vi "test_Set and Get 9227.vi"(8 "error in (no error)":errorcluster, 11 "TestCase in":refnum<class "Scan Engine Scripting API Custom Device Unit Tests.lvclass">) -> (0 "error out":errorcluster, 3 "TestCase out":refnum<class "Scan Engine Scripting API Custom Device Unit Tests.lvclass">)   [LabVIEW 2027, in "Scan Engine Scripting API Custom Device Unit Tests.lvclass"]
uses:
  Scan Engine Scripting API Custom Device Unit Tests.lvclass
  Scan Engine Scripting API Custom Device Unit Tests.lvclass/Scan Engine Scripting API Custom Device Unit Tests.ctl
  Scripting/Modules/NI 9227/NI 9227.lvclass
  C:/NetCore/niveristand-scan-engine-ethercat-custom-device/Custom Device Source/Scripting/Modules/Module/Module.lvclass
  C:/NetCore/niveristand-scan-engine-ethercat-custom-device/Custom Device Source/Scripting/Modules/NI 9227/NI 9227.lvclass
  C:/Program Files/National Instruments/LabVIEW 2027/vi.lib/addons/_JKI Toolkits/VI Tester/TestCase.llb/TestCase.lvclass
  C:/NetCore/niveristand-scan-engine-ethercat-custom-device/Custom Device Source/Tests/Unit Tests/Scripting API/Custom Device/Scan Engine Scripting API Custom Device Unit Tests.lvclass
  <vilib>/addons/_JKI Toolkits/VI Tester/TestCase.llb/TestCase.lvclass
  Scripting/Scan Engine Scripting.lvlib
  b7875b56-ce47-4e38-ae1e-efee4344b8b5.vi
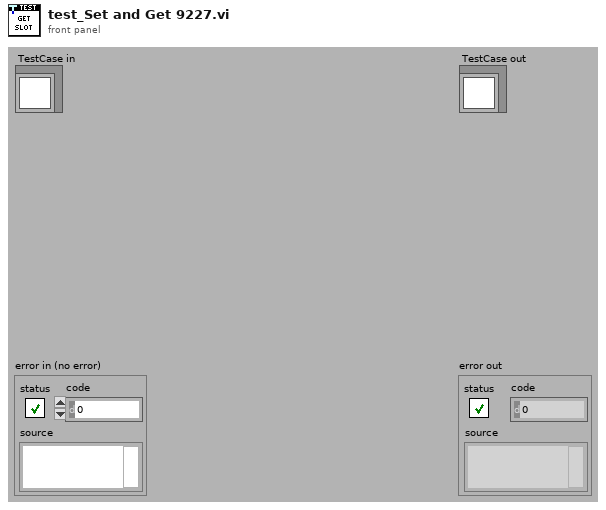
[diagram p1: front panel]
types:
  T1 = typedef "Custom Device API.lvlib/Custom Device Item Ref.ctl" = u64
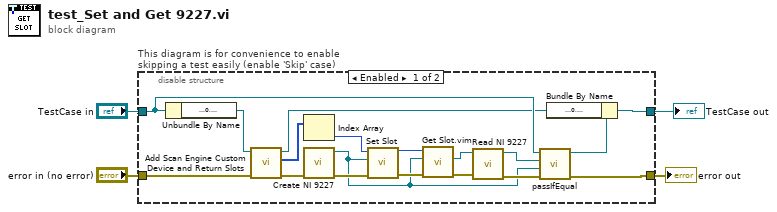
[diagram p0: block diagram]
diagram:
  n1 = disable-structure "This diagram is for convenience to enable skipping a test easily (enable 'Skip' case)" shown="Enabled" {
    disable-tunnel: "TestCase in" -> [w17 w26]
    disable-tunnel: [w18 w24] -> w1
    disable-tunnel: [w12 w25] -> w3
    disable-tunnel: "error in (no error)" -> [w22 w23]
    frame Enabled {
      n2 = Unbundle By Name(w17) -> ("target ref"=w21:refnum<k24>)
      n3 = call "Add Scan Engine Custom Device and Return Slots.vi"("error in"=w22, "target ref in"=w21) -> ("error out"=w15:errorcluster, "slot refs"=w20:T1[], "target ref out"=w16:refnum<k24>)  [unwired: 7 in]
      n4 = Index Array(array=w20) -> (element=w19:T1)  [unwired: 1 in]
      n5 = call "Create NI 9227.vi"("error in"=w15) -> ("error out"=w14:errorcluster, "NI 9227 out"=w7:refnum<class "NI 9227.lvclass">)  [unwired: 9 in]
      n6 = call "Set Slot.vi"("error in"=w14, "module"=w7, "slot ref in"=w19) -> ("error out"=w8:errorcluster, "slot ref out"=w5:T1)  [unwired: 7 in]
      n7 = call "Get Slot.vim"("error in"=w8, "module type"=w7, "slot ref in"=w5) -> ("error out"=w13:errorcluster, "module"=w6:refnum<class "NI 9227.lvclass">)  [unwired: 5 in, 2 out]
      n8 = call "Read NI 9227.vi"("error in"=w13, "NI 9227 in"=w6) -> ("error out"=w10:errorcluster, "NI 9227 out"=w11:refnum<class "NI 9227.lvclass">)  [unwired: 7 in, 1 out]
      n9 = call-dynamic "passIfEqual.vi"("error in (no error)"=w10, "y"=w7, "x"=w11, "TestCase in"=w17) -> ("error out"=w12:errorcluster, "TestCase out"=w9:refnum<class "Scan Engine Scripting API Custom Device Unit Tests.lvclass">)  [unwired: 6 in]
      n10 = Bundle By Name(cluster=w9, "target ref"=w16) -> (w18:refnum<class "Scan Engine Scripting API Custom Device Unit Tests.lvclass">)
    }
    frame Disabled {
      # "skip test result while test is under development"
      n11 = call <vilib>:"skip.vi"("error in (no error)"=w23, "TestCase in"=w26) -> ("error out"=w25:errorcluster, "TestCase out"=w24:refnum<class "Scan Engine Scripting API Custom Device Unit Tests.lvclass">)  [unwired: 8 in]
    }
  }
  "error out" <- w3
  "TestCase out" <- w1
